vi "VIH HelpGen - FILE - Build Relative Path.vi"(5 "Don't convert to relative (F)":bool, 7 "Root Path":path, 10 "Allow Empty Path (T)":bool=TRUE, 11 "Path in":path) -> (3 "Path out":path)   [LabVIEW 2014]
doc: "::: VI Helpeks :::\nCopyright (c) 2000-2026 Konstantin Shifershteyn. All rights reserved."
panel:
  # "VI Helpeks\nCopyright (c) 2012-2026 Konstantin Shifershteyn"
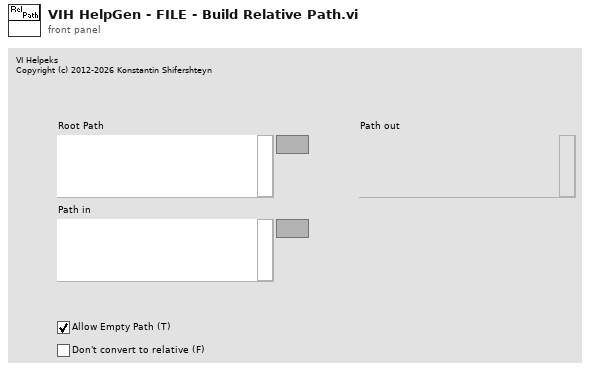
[diagram p1: front panel]
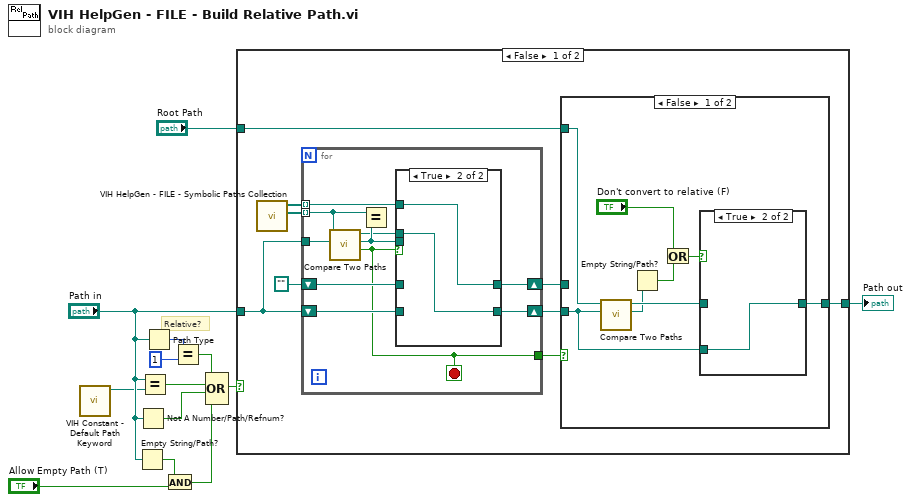
[diagram p0: block diagram]
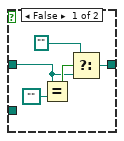
[diagram p2: hidden frame]
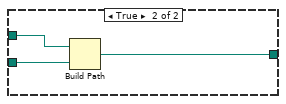
[diagram p3: hidden frame]
diagram:
  # "Relative?"
  n1 = call "VIH Constant - Default Path Keyword.vi"() -> ("<default> path"=w2:path)  [unwired: 11 in]
  n2 = Empty String/Path?(string/path="Path in") -> (empty?=w5:bool)
  n3 = Not A Number/Path/Refnum?(number/path/refnum="Path in") -> (NaN/Path/Refnum?=w7:bool)
  n4 = Equal?(x="Path in", y=w2) -> (x = y?=w8:bool)
  n5 = Path Type(1:"Path in") -> (0:w11:i16)
  n6 = And(x=w5, y="Allow Empty Path (T)") -> (x .and. y?=w3:bool)
  n7 = Equal?(x=w11, y=i16 1) -> (x = y?=w9:bool)
  n8 = Compound Arithmetic op=OR(w9, w8, w7, w3) -> (w1:bool)
  n9 = case shown="False" w1 {
    tunnel: "Path in" -> [w22 w54]
    tunnel: [w16 w54] -> w13
    tunnel: "Root Path" -> [w15 _]
    frame False {
      n10 = call "VIH HelpGen - FILE - Symbolic Paths Collection.vi"() -> ("Absolute Paths"=w17:path[], "Symbolic Paths"=w18:path[])  [unwired: 10 in]
      n11 = for {
        tunnel: w17 -> [w49] mode=indexing
        tunnel: w22 -> [w48]
        shift-right: [w47] -> w20
        shift-left: path "" -> [w46]
        shift-right: [w45] -> w19
        shift-left: w22 -> [w44]
        tunnel: w18 -> [w42] mode=indexing
        tunnel: [w40] -> w14
        stop <- w40 stop-if-true
        n12 = call <vilib>:"Compare Two Paths.vi"("Path 2"=w48, "Path 1"=w49) -> ("Path 2 Relative to Path 1?"=w40:bool, "Common Path"=w43:path, "Relative Path from 1 to 2"=w41:path)  [unwired: 6 in, 1 out]
        n13 = Equal?(x=w49, y=w43) -> ()  [unwired: 1 out]
        n14 = case shown="True" w40 {
          tunnel: [w51 w53] -> w47
          tunnel: w46 -> [w51 _]
          tunnel: [w50 w52] -> w45
          tunnel: w44 -> [w50 _]
          tunnel: w43 -> [_ _]
          tunnel: w42 -> [_ w53]
          tunnel: w41 -> [_ w52]
          frame False {
          }
          frame True {
          }
        }
      }
      n15 = case shown="False" w14 {
        tunnel: w20 -> [_ w39]
        tunnel: w19 -> [w26 w38]
        tunnel: [w29 w37] -> w16
        tunnel: w15 -> [w30 _]
        frame False {
          n16 = call <vilib>:"Compare Two Paths.vi"("Path 2"=w26, "Path 1"=w30) -> ("Common Path"=w27:path, "Relative Path from 1 to 2"=w28:path)  [unwired: 6 in, 2 out]
          n17 = Empty String/Path?(string/path=w27) -> (empty?=w25:bool)
          n18 = Or(x="Don't convert to relative (F)", y=w25) -> (x .or. y?=w24:bool)
          n19 = case shown="True" w24 {
            tunnel: [w34 w36] -> w29
            tunnel: w28 -> [w31 _]
            tunnel: w26 -> [_ w36]
            frame False {
              n20 = Equal?(x=w31, y=path "" ("x")) -> (x = y?=w35:bool)
              n21 = Select(t=path "", s=w35, f=w31) -> (s? t:f=w34:path)
            }
            frame True {
            }
          }
        }
        frame True {
          n22 = Build Path(base path=w39, name or relative path=w38) -> (appended path=w37:path)
        }
      }
    }
    frame True {
    }
  }
  "Path out" <- w13
